vi "Finish Sequence.vi"(8 "error in":errorcluster, 11 "Sequence Executor in":refnum<class "Sequence Executor.lvclass">) -> (0 "error out":errorcluster, 3 "Sequence Executor out":refnum<class "Sequence Executor.lvclass">)   [LabVIEW 2026, in "Sequence Executor.lvclass"]
doc: "Helper, called after the last step. Running false, Phase Idle, Overall Verdict PASS when every step result equals its expected_result else FAIL, CSV report written to Results Folder, plant driven to safe setpoints 0, 0, 0, Status COMPLETE with verdict and report path. A CSV write error is shown in Status and NOT returned."
uses:
  Sequence Executor.lvclass
  Sequence Executor.lvclass/Sequence Executor.ctl
  C:/Program Files/National Instruments/LabVIEW 2026/vi.lib/ActorFramework/Actor/Actor.lvclass
  C:/Users/DynaAdmin/PycharmProjects/Universal-sequence-executor-AF/src/Executor/Sequence Executor.lvclass
  <vilib>/ActorFramework/Message Enqueuer/Message Enqueuer.lvclass
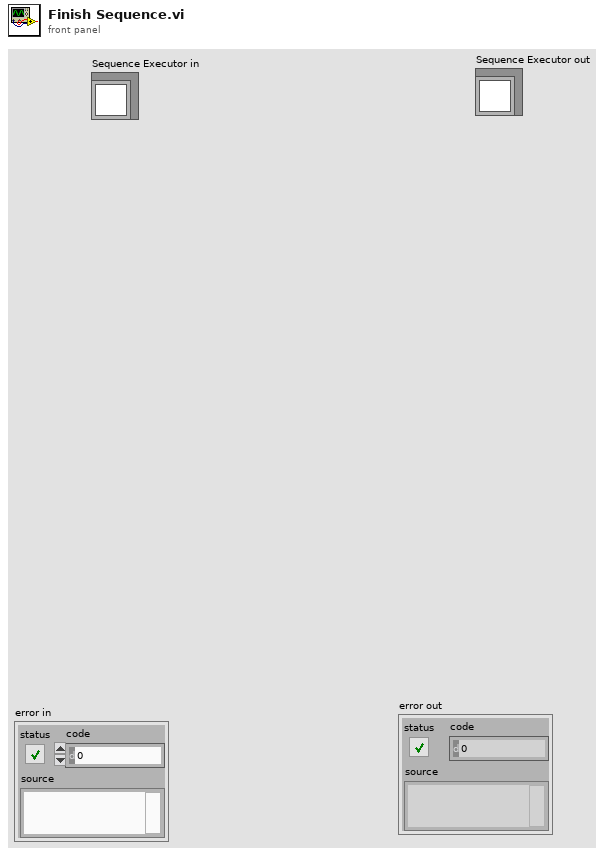
[diagram p1: front panel]
types:
  T1 = cluster{"pressure_sp_bar":dbl, "flow_sp_lpm":dbl, "displacement_sp_mm":dbl}
  T2 = typedef "Sequence File.ctl" = cluster{"sequence_id":string, "description":string, "total_steps":i32, "steps":T3[]}
  T3 = typedef "Step Config.ctl" = cluster{"step_no":i32, "step_name":string, "command_type":string, "pressure_sp_bar":dbl, "flow_sp_lpm":dbl, "displacement_sp_mm":dbl, "monitored_io":string, "tolerance_bar":dbl, "dwell_time_ms":i32, "timeout_ms":i32, "expected_result":string}
  T4 = typedef "Step Result.ctl" = cluster{"step_no":i32, "step_name":string, "result":string, "reason":string, "measured":dbl, "target":dbl, "duration_ms":dbl}
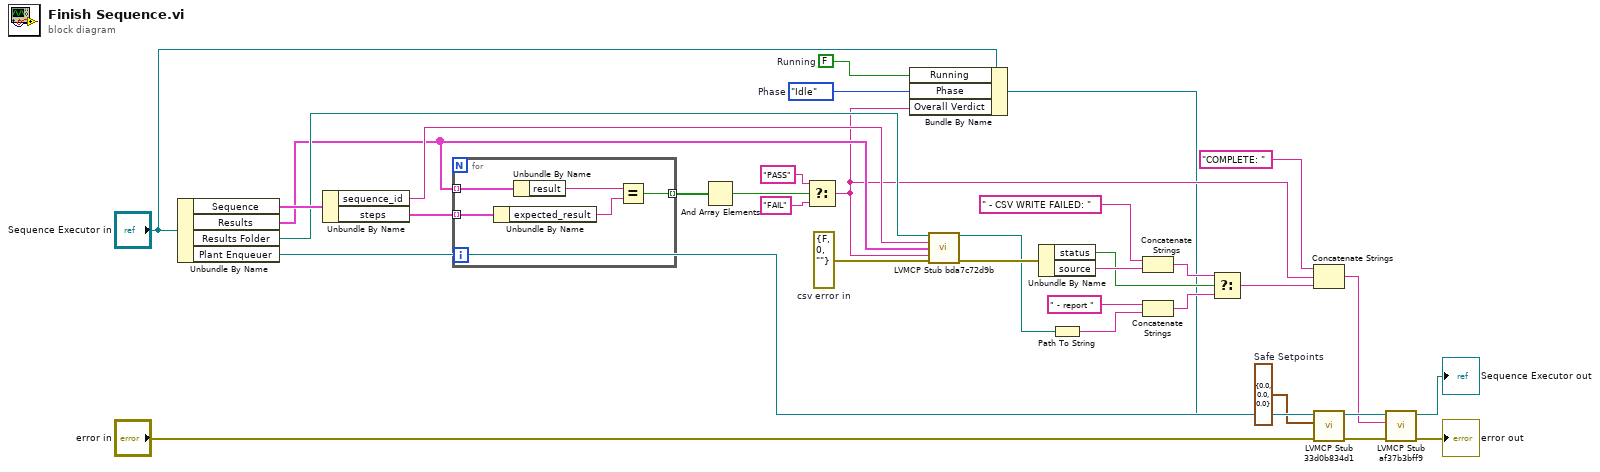
[diagram p0: block diagram]
diagram:
  w7 = T1 {"pressure_sp_bar"=0.0, "flow_sp_lpm"=0.0, "displacement_sp_mm"=0.0}  # Safe Setpoints
  w11 = enum16{"Idle", "Settling", "Dwell", "Complete"}."Idle"  # Phase
  w12 = FALSE  # Running
  w24 = errorcluster {"status"=FALSE, "code"=0, "source"=""}  # csv error in
  n1 = Unbundle By Name("Sequence Executor in") -> ("Sequence"=w33:T2, "Results"=w25:T4[], "Results Folder"=w27:path, "Plant Enqueuer"=w8:refnum<class "Message Enqueuer.lvclass">)
  n2 = Unbundle By Name(w33) -> ("sequence_id"=w26:string, "steps"=w32:T3[])
  n3 = for {
    tunnel: w25 -> [w38] mode=indexing
    tunnel: w32 -> [w37] mode=indexing
    tunnel: [w34] -> w31 mode=indexing
    n4 = Unbundle By Name(w37) -> ("expected_result"=w35:string)
    n5 = Unbundle By Name(w38) -> ("result"=w36:string)
    n6 = Equal?(x=w36, y=w35) -> (x = y?=w34:bool)
  }
  n7 = And Array Elements(Boolean array=w31) -> (logical AND=w29:bool)
  n8 = Select(t="PASS", s=w29, f="FAIL") -> (s? t:f=w10:string)
  n9 = Bundle By Name(cluster="Sequence Executor in", "Running"=w12, "Phase"=w11, "Overall Verdict"=w10) -> (w5:refnum<class "Sequence Executor.lvclass">)
  n10 = call <userlib>:"LVMCP Stub bda7c72d9b.vi"("results folder path"=w27, "sequence_id"=w26, "Step Results"=w25, "overall verdict"=w10, "error in"=w24) -> ("file path"=w22:path, "error out"=w23:errorcluster)  [unwired: 9 in]
  n11 = Unbundle By Name(w23) -> ("status"=w16:bool, "source"=w20:string)
  n12 = Path To String(path=w22) -> (string=w18:string)
  n13 = Concatenate Strings(" - CSV WRITE FAILED: ", w20) -> (w17:string)
  n14 = Concatenate Strings(" - report ", w18) -> (w15:string)
  n15 = Select(t=w17, s=w16, f=w15) -> (s? t:f=w13:string)
  n16 = Concatenate Strings("COMPLETE: ", w10, w13) -> (w4:string)
  n17 = call <userlib>:"LVMCP Stub 33d0b834d1.vi"("error in (no error)"="error in", "Plant Setpoints"=w7, "Message Enqueuer"=w8) -> ("error out"=w3:errorcluster)  [unwired: 7 in, 1 out]
  n18 = call <userlib>:"LVMCP Stub af37b3bff9.vi"("error in"=w3, "Status"=w4, "Sequence Executor in"=w5) -> ("error out"=→"error out":errorcluster, "Sequence Executor out"=→"Sequence Executor out":path)  [unwired: 7 in]
